vi "Update Control from Metadata.vi"(6 "default_value":variant, 8 "error in":errorcluster, 9 "control name":string, 10 "parameter data":T1[](array[typedef]), 11 "vi refnum in":refnum<vi>) -> (0 "error out":errorcluster, 3 "vi refnum out":refnum<vi>)   [LabVIEW 2021, in "NI Measurement V2 Client Generator Runtime.lvlib"]
uses:
  NI Measurement V2 Client Generator Runtime.lvlib
  <vilib>/gRPC/Generated APIs/ni/measurementlink/measurement/v2/Measurement Service Client V2/RPC Messages/ni_measurementlink_measurement_v2_ConfigurationParameter.ctl
  <vilib>/gRPC/Generated APIs/ni/measurementlink/measurement/v2/Measurement Service Client V2/RPC Messages/google_protobuf_Field_Kind.ctl
  <vilib>/gRPC/Generated APIs/ni/measurementlink/measurement/v2/Measurement Service Client V2/RPC Messages/ni_measurementlink_measurement_v2_ConfigurationParameter_AnnotationsEntry.ctl
  <vilib>/Utility/miscctls.llb/LVPositionTypeDef.ctl
  Client Generator Error Strings Global.vi
  <vilib>/gRPC/Generated APIs/ni/measurementlink/measurement/v2/Measurement Service Client V2/Measurement Service Client V2.lvlib
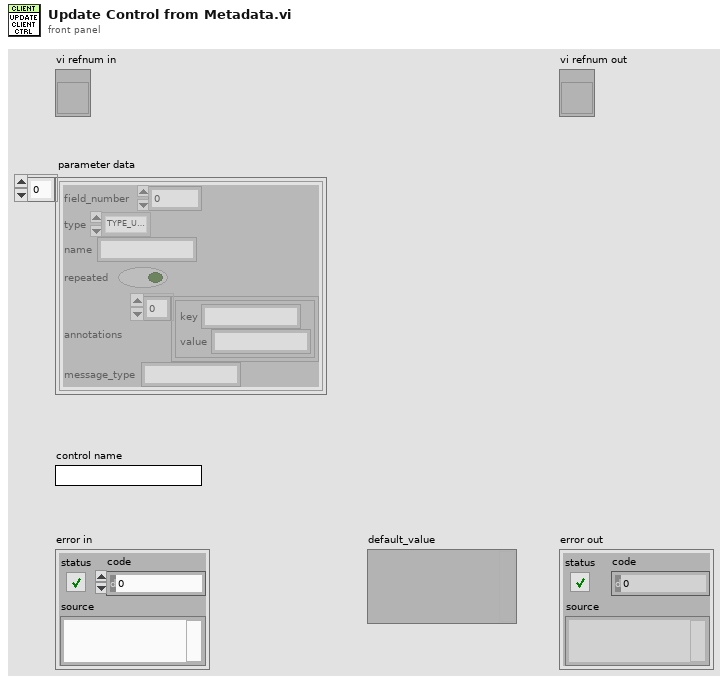
[diagram p1: front panel]
types:
  T1 = typedef "Measurement Service Client V2.lvlib/ni_measurementlink_measurement_v2_ConfigurationParameter.ctl" = cluster{"field_number":i32, "type":T2, "name":string, "repeated":bool, "annotations":T3[], "message_type":string}
  T2 = typedef "Measurement Service Client V2.lvlib/google_protobuf_Field_Kind.ctl" = enum32{"TYPE_UNKNOWN", "TYPE_DOUBLE", "TYPE_FLOAT", "TYPE_INT64", "TYPE_UINT64", "TYPE_INT32", "TYPE_FIXED64", "TYPE_FIXED32", "TYPE_BOOL", "TYPE_STRING", "TYPE_GROUP", "TYPE_MESSAGE", "TYPE_BYTES", "TYPE_UINT32", "TYPE_ENUM", "TYPE_SFIXED32", "TYPE_SFIXED64", "TYPE_SINT32", "TYPE_SINT64"}
  T3 = typedef "Measurement Service Client V2.lvlib/ni_measurementlink_measurement_v2_ConfigurationParameter_AnnotationsEntry.ctl" = cluster{"key":string, "value":string}
  T4 = typedef "LVPositionTypeDef.ctl" = cluster{"Left":i32, "Top":i32}
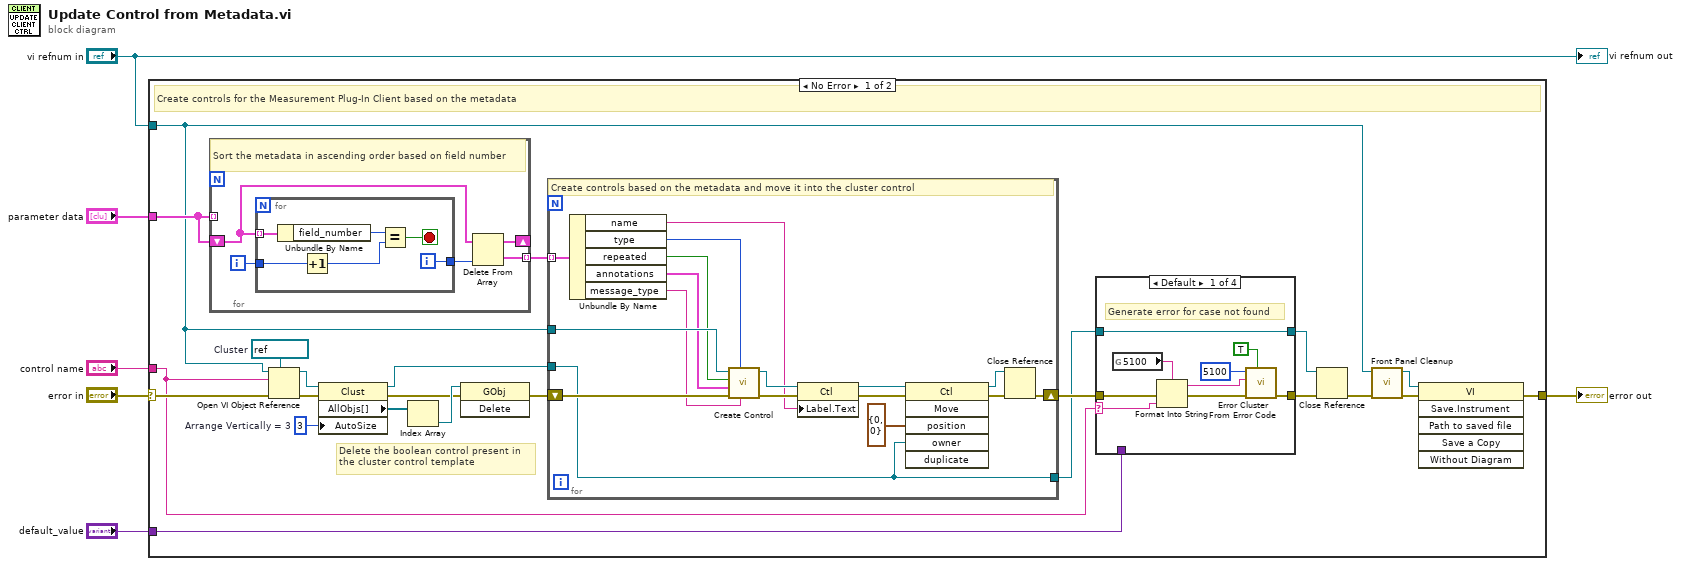
[diagram p0: block diagram]
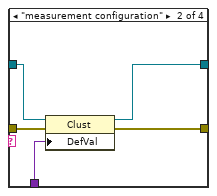
[diagram p2: hidden frame]
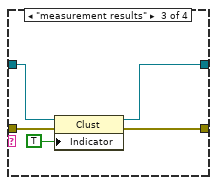
[diagram p3: hidden frame]
diagram:
  n1 = case shown="No Error" "error in" {
    selector: "error in" -> [w23 w79]
    tunnel: "control name" -> [w16 _]
    tunnel: "parameter data" -> [w14 _]
    tunnel: "vi refnum in" -> [w9 _]
    tunnel: [w7 w79] -> w4
    tunnel: "default_value" -> [w12 _]
    frame No Error {
      w22 = u32 3  # Arrange Vertically = 3
      w29 = refnum<vi> refnum  # Cluster
      # "Delete the boolean control present in\nthe cluster control template"
      # "Create controls for the Measurement Plug-In Client based on the metadata"
      n2 = for {
        shift-right: [w48] -> _
        shift-left: w14 -> [w49]
        tunnel: [w47] -> w15 mode=indexing
        tunnel: w14 -> [_] mode=indexing
        i -> [w51]
        # "Sort the metadata in ascending order based on field number"
        n3 = for {
          tunnel: w49 -> [w54] mode=indexing
          tunnel: w51 -> [w57]
          tunnel: [w53] -> w50
          i -> [w53]
          stop <- w52 stop-if-true
          n4 = Unbundle By Name(w54) -> ("field_number"=w56:i32)
          n5 = Increment(x=w57) -> (x+1=w55:i32)
          n6 = Equal?(x=w56, y=w55) -> (x = y?=w52:bool)
        }
        n7 = Delete From Array(array=w49, index=w50) -> (deleted portion=w47:T1, array with subset deleted=w48:T1[])  [unwired: 1 in]
      }
      n8 = Open VI Object Reference(7:w29, 8:w23, 10:w16, 11:w9) -> (0:w27:errorcluster, 3:w28:refnum<vi>)
      n9 = property class="Clust"(reference=w28, error in=w27, "AutoSize"=w22) -> (reference out=w19:refnum<vi>, error out=w24:errorcluster, "AllObjs[]"=w26:refnum<vi>[])
      n10 = Index Array(array=w26) -> (element=w25:refnum<vi>)  [unwired: 1 in]
      n11 = invoke class="GObj" method="Delete"(reference=w25, error in=w24) -> (error out=w21:errorcluster)  [unwired: 1 in, 2 out]
      n12 = for {
        shift-right: [w34] -> w20
        shift-left: w21 -> [w46]
        tunnel: w9 -> [w44]
        tunnel: w19 -> [w32]
        tunnel: [w32] -> w17
        tunnel: w15 -> [w30] mode=indexing
        # "Create controls based on the metadata and move it into the cluster control"
        n13 = Unbundle By Name(w30) -> ("name"=w38:string, "type"=w42:T2, "repeated"=w43:bool, "annotations"=w41:T3[], "message_type"=w40:string)
        n14 = call "Create Control.vi"("message_type"=w40, "type"=w42, "error in"=w46, "annotations"=w41, "is repeated?"=w43, "vi refnum"=w44) -> ("error out"=w45:errorcluster, "control ref"=w39:refnum<vi>)  [unwired: 4 in]
        n15 = property class="Ctl"(reference=w39, error in=w45, "Label.Text"=w38) -> (reference out=w37:refnum<vi>, error out=w36:errorcluster)
        n16 = invoke class="Ctl" method="Move"(reference=w37, error in=w36, "position"=T4 {"Left"=0, "Top"=0}, "owner"=w32) -> (reference out=w33:refnum<vi>, error out=w35:errorcluster)  [unwired: 2 in, 4 out]
        n17 = Close Reference(reference=w33, error in (no error)=w35) -> (error out=w34:errorcluster)
      }
      n18 = case shown="Default" w16 {
        selector: w16 -> [w61 _ _ _]
        tunnel: w20 -> [w66 w71 w76 w77]
        tunnel: [w64 w70 w75 w77] -> w18
        tunnel: w17 -> [w65 w69 w74 w78]
        tunnel: [w65 w68 w73 w78] -> w11
        tunnel: w12 -> [_ w67 _ _]
        frame Default {
          # "Generate error for case not found"
          n19 = global read "Client Generator Error Strings Global.vi" "5100"() -> (w58:string)
          n20 = Format Into String(format string=w58, error in=w66, w61) -> (resulting string=w59:string, error out=w62:errorcluster)  [unwired: 1 in]
          n21 = call <vilib>:"Error Cluster From Error Code.vi"("show call chain? (False)"=TRUE, "error in (no error)"=w62, "error message (\"\")"=w59, "error code (0)"=5100) -> ("error out"=w64:errorcluster)  [unwired: 5 in]
        }
        frame "measurement configuration" {
          n22 = property class="Clust"(reference=w69, error in=w71, "DefVal"=w67) -> (reference out=w68:refnum<vi>, error out=w70:errorcluster)
        }
        frame "measurement results" {
          n23 = property class="Clust"(reference=w74, error in=w76, "Indicator"=TRUE) -> (reference out=w73:refnum<vi>, error out=w75:errorcluster)
        }
        frame "configuration" {
        }
      }
      n24 = Close Reference(reference=w11, error in (no error)=w18) -> (error out=w13:errorcluster)
      n25 = call "Front Panel Cleanup.vi"("error in"=w13, "vi refnum"=w9) -> ("error out"=w10:errorcluster, "vi refnum out"=w8:refnum<vi>)  [unwired: 8 in]
      n26 = invoke class="VI" method="Save.Instrument"(reference=w8, error in=w10) -> (error out=w7:errorcluster)  [unwired: 4 in, 5 out]
    }
    frame Error {
      # "Pass"
    }
  }
  "error out" <- w4
  "vi refnum out" <- "vi refnum in"
